vi "Run.vi"() -> ()   [LabVIEW 2019]
uses:
  App/Generic Test Stand/Generic Test Stand.lvclass
  App/Generic Test Stand/Generic Test Stand.lvclass/Generic Test Stand.ctl
  App/TS Framework/TS Framework.lvlib
panel:
  in  "Cryo Sep":bool caption="Button"
  in  "DeepU":bool caption="Button"
  in  "LNG Boiling":bool caption="Button"
  in  "Water Tunnel":bool caption="Button"
  in  "Heat Flow":bool caption="Button"
  in  "HTS":bool caption="Button"
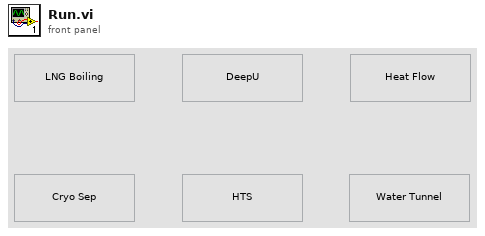
[diagram p1: front panel]
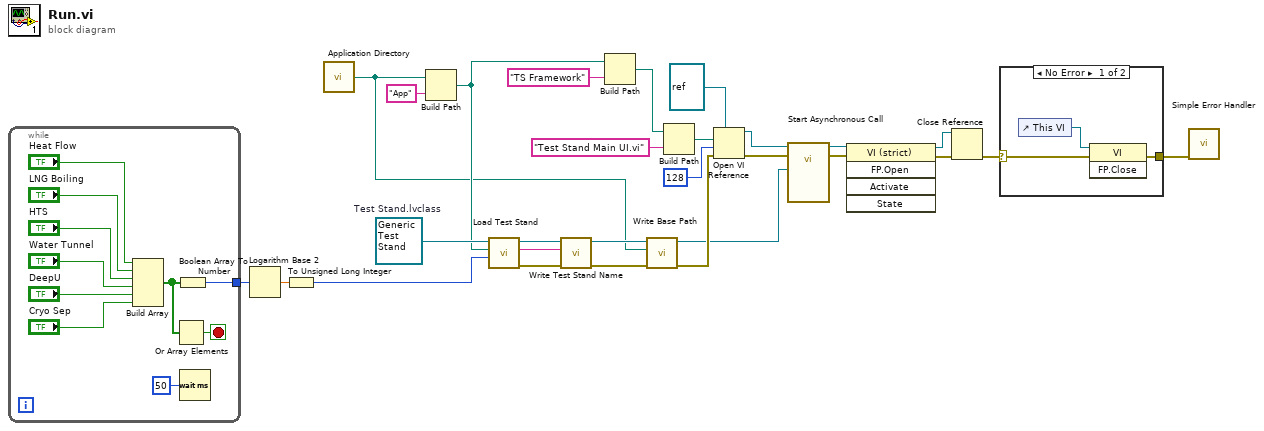
[diagram p0: block diagram]
diagram:
  w28 = refnum<class "Generic Test Stand.lvclass"> refnum  # Test Stand.lvclass
  n1 = while {
    tunnel: [w35] -> w25
    stop <- w37 stop-if-true
    n2 = Build Array("Heat Flow", "LNG Boiling", "HTS", "Water Tunnel", "DeepU", "Cryo Sep") -> (w36:bool[])
    n3 = Or Array Elements(Boolean array=w36) -> (logical OR=w37:bool)
    n4 = Boolean Array To Number(Boolean array=w36) -> (number=w35:u32)
    n5 = Wait (ms)(milliseconds to wait=u32 50) -> ()  [unwired: 1 out]
  }
  n6 = Logarithm Base 2(1:w25) -> (0:w24:dbl)
  n7 = To Unsigned Long Integer(number=w24) -> (unsigned 32bit integer=w9:u32)
  n8 = call <vilib>:"Application Directory.vi"() -> ("Application Directory"=w1:path)
  n9 = Build Path(base path=w1, name or relative path="App") -> (appended path=w26:path)
  n10 = call "Load Test Stand.vi"("Select Test Stand"=w9, "App Base Path"=w26, "Test Stand.lvclass"=w28) -> ("Error Out"=w7:errorcluster, "Test Stand Name"=w2:string, "Specific Test Stand.lvclass"=w8:refnum<class "Generic Test Stand.lvclass">)  [unwired: 6 in]
  n11 = call "Write Test Stand Name.vi"("error in (no error)"=w7, "Test Stand Name"=w2, "Generic Test Stand in"=w8) -> ("error out"=w5:errorcluster, "Generic Test Stand out"=w6:refnum<class "Generic Test Stand.lvclass">)  [unwired: 7 in]
  n12 = Build Path(base path=w26, name or relative path="TS Framework") -> (appended path=w11:path)
  n13 = call "Write Base Path.vi"("error in (no error)"=w5, "Base Path"=w1, "Generic Test Stand in"=w6) -> ("error out"=w4:errorcluster, "Generic Test Stand out"=w3:refnum<class "Generic Test Stand.lvclass">)  [unwired: 7 in]
  n14 = Build Path(base path=w11, name or relative path="Test Stand Main UI.vi") -> (appended path=w18:path)
  n15 = Open VI Reference(type specifier VI Refnum (for type only)=refnum<vi> refnum, vi path=w18, options=128, error in (no error)=w4) -> (vi reference=w20:refnum<vi>, error out=w19:errorcluster)  [unwired: 2 in]
  n16 = call-by-ref "Start Asynchronous Call"(reference=w20, error in=w19, "Test Stand.lvclass"=w3) -> (reference out=w17:refnum<vi>, error out=w15:errorcluster)  [unwired: 11 in]
  n17 = invoke class="VI (strict)" method="FP.Open"(reference=w17, error in=w15) -> (reference out=w16:refnum<vi>, error out=w14:errorcluster)  [unwired: 3 in, 3 out]
  n18 = Close Reference(reference=w16, error in (no error)=w14) -> (error out=w13:errorcluster)
  n19 = case shown="No Error" w13 {
    selector: w13 -> [w40 w42]
    tunnel: [w39 w42] -> w10
    frame No Error {
      n20 = control-ref of="This VI"() -> (w41:refnum<vi>)
      n21 = invoke class="VI" method="FP.Close"(reference=w41, error in=w40) -> (error out=w39:errorcluster)  [unwired: 1 in, 2 out]
    }
    frame Error {
    }
  }
  n22 = call <vilib>:"Simple Error Handler.vi"("error in (no error)"=w10) -> ()  [unwired: 4 in, 5 out]
